vi "GlobalesPrensa.vi"() -> ()   [LabVIEW 2026]
panel:
  in  "tQX":dbl
  in  "F_QX":dbl
  in  "Salir":bool
  in  "ArchivoControl":path=path "D:/2026/control_sin_registro.csv"
  in  "InfoEnsayo":string="ASTM 1609 con100x100x350"
  in  "Ensayando":bool
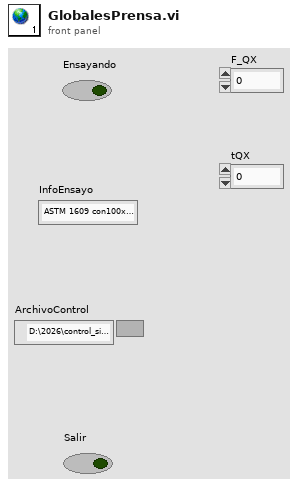
[diagram p1: front panel]
diagram:
